vi "Keys_Apply.vi"(0 "State":T1={"Tick"=0, "Phase"=0, "PhaseTicks"=0, "Level"=1, "Room"=0, "X10"=0, "Y10"=0, "VY10"=0, "Mode"=0, "Facing"=0, "Run"=0, "Vert"=0, "StandY"=0, "EntryX10"=0, "EntryY10"=0, "EntryMode"=0, "Lives"=4, "Score"=0, "NextLife"=10000, "KeyR"=0, "KeyB"=0, "KeyY"=0, "Torch"=FALSE, "FloorPhase"=0, "Dead"=FALSE, "LevelStart"=FALSE, "Quit"=FALSE, "Sound"=0, "Seed"=12345, "DemoStep"=0, "Tiles"=[], "World"=[], "Enemies"=[], "Highscores"=[], "Name"=[0, 0, 0], "Cursor"=0}, 5 "Key":u16, 11 "error in":errorcluster) -> (4 "State out":T1={"Tick"=0, "Phase"=0, "PhaseTicks"=0, "Level"=1, "Room"=0, "X10"=0, "Y10"=0, "VY10"=0, "Mode"=0, "Facing"=0, "Run"=0, "Vert"=0, "StandY"=0, "EntryX10"=0, "EntryY10"=0, "EntryMode"=0, "Lives"=4, "Score"=0, "NextLife"=10000, "KeyR"=0, "KeyB"=0, "KeyY"=0, "Torch"=FALSE, "FloorPhase"=0, "Dead"=FALSE, "LevelStart"=FALSE, "Quit"=FALSE, "Sound"=0, "Seed"=12345, "DemoStep"=0, "Tiles"=[], "World"=[], "Enemies"=[], "Highscores"=[], "Name"=[0, 0, 0], "Cursor"=0}, 15 "error out":errorcluster)   [LabVIEW 2020, in "GH_Engine.lvlib"]
doc: "Applies a key to the movement wishes: Left/Right set Run, ReleaseL/ReleaseR stop only the matching direction, Release stops, Up/Down set Vert, ReleaseV stops climbing."
uses:
  GH_Engine.lvlib
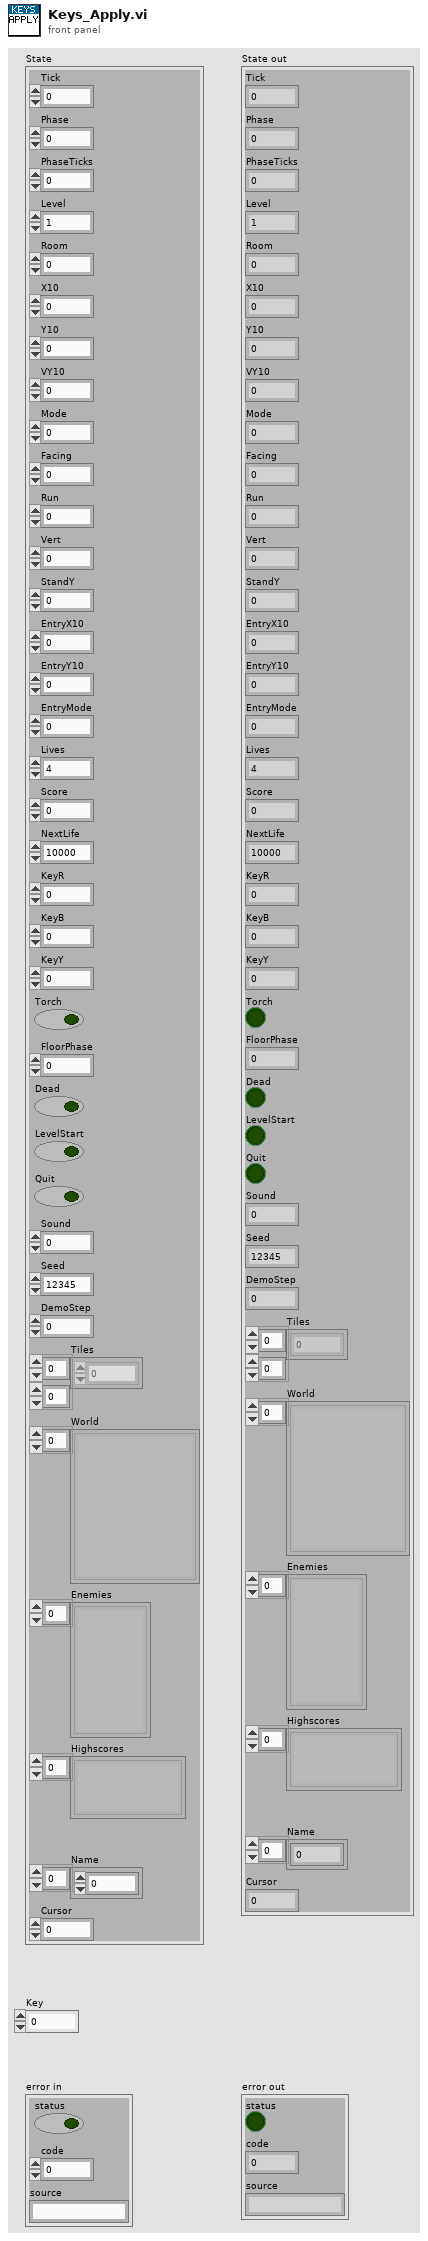
[diagram p1: front panel]
types:
  T1 = cluster{"Tick":u32, "Phase":i32, "PhaseTicks":i32, "Level":i32, "Room":i32, "X10":i32, "Y10":i32, "VY10":i32, "Mode":i32, "Facing":i32, "Run":i32, "Vert":i32, "StandY":i32, "EntryX10":i32, "EntryY10":i32, "EntryMode":i32, "Lives":i32, "Score":i32, "NextLife":i32, "KeyR":i32, "KeyB":i32, "KeyY":i32, "Torch":bool, "FloorPhase":i32, "Dead":bool, "LevelStart":bool, "Quit":bool, "Sound":i32, "Seed":u32, "DemoStep":i32, "Tiles":u8[][], "World":cluster{"ID":string, "Depth":i32, "Column":i32, "Tiles":u8[][]}[], "Enemies":cluster{"Kind":i32, "X10":i32, "Y10":i32, "Dir":i32, "Mode":i32}[], "Highscores":cluster{"Score":i32, "Name":string}[], "Name":i32[], "Cursor":i32}
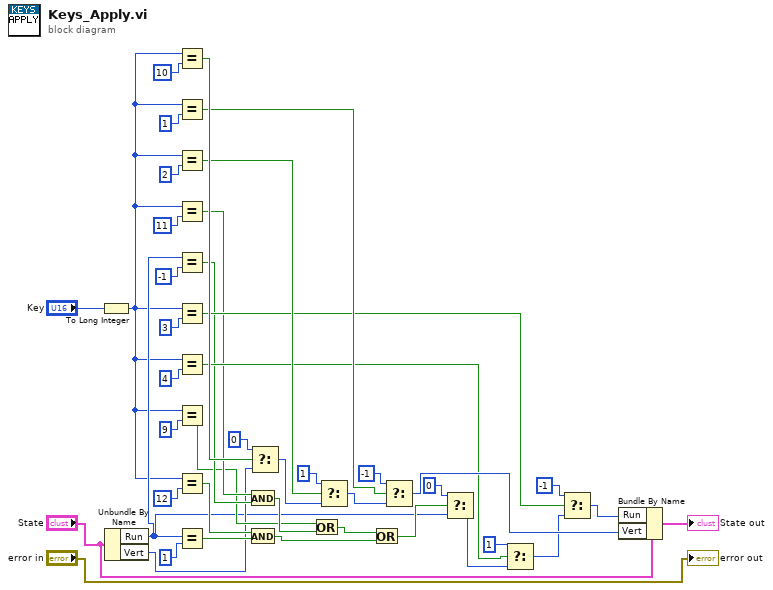
[diagram p0: block diagram]
diagram:
  n1 = To Long Integer(number="Key") -> (32bit integer=w4:i32)
  n2 = Unbundle By Name("State") -> ("Run"=w5:i32, "Vert"=w6:i32)
  n3 = Equal?(x=w4, y=10) -> (x = y?=w38:bool)
  n4 = Equal?(x=w4, y=1) -> (x = y?=w32:bool)
  n5 = Equal?(x=w4, y=2) -> (x = y?=w35:bool)
  n6 = Equal?(x=w4, y=11) -> (x = y?=w10:bool)
  n7 = Equal?(x=w5, y=-1) -> (x = y?=w12:bool)
  n8 = Equal?(x=w4, y=3) -> (x = y?=w22:bool)
  n9 = Equal?(x=w4, y=4) -> (x = y?=w25:bool)
  n10 = Equal?(x=w4, y=9) -> (x = y?=w8:bool)
  n11 = Equal?(x=w4, y=12) -> (x = y?=w15:bool)
  n12 = Equal?(x=w5, y=1) -> (x = y?=w17:bool)
  n13 = And(x=w10, y=w12) -> (x .and. y?=w13:bool)
  n14 = And(x=w15, y=w17) -> (x .and. y?=w18:bool)
  n15 = Select(t=0, s=w38, f=w6) -> (s? t:f=w40:i32)
  n16 = Or(x=w8, y=w13) -> (x .or. y?=w19:bool)
  n17 = Select(t=1, s=w35, f=w40) -> (s? t:f=w41:i32)
  n18 = Or(x=w19, y=w18) -> (x .or. y?=w20:bool)
  n19 = Select(t=-1, s=w32, f=w41) -> (s? t:f=w42:i32)
  n20 = Select(t=0, s=w20, f=w5) -> (s? t:f=w28:i32)
  n21 = Select(t=1, s=w25, f=w28) -> (s? t:f=w29:i32)
  n22 = Select(t=-1, s=w22, f=w29) -> (s? t:f=w30:i32)
  n23 = Bundle By Name(cluster="State", "Run"=w30, "Vert"=w42) -> (→"State out":T1)
  "error out" <- "error in"
